vi "HostMem Reshape.vi"(4 "rows":i32, 6 "cn":i32, 8 "error in (no error)":errorcluster, 11 "HostMem in":refnum<class "HostMem.lvclass">) -> (0 "error out":errorcluster, 2 "Dst out":refnum<class "HostMem.lvclass">, 3 "HostMem out":refnum<class "HostMem.lvclass">)   [LabVIEW 2020, in "OpenLvVision_OpenCv.lvlib" / "Cuda.lvlib" / "HostMem.lvclass"]
doc: "creates alternative HostMem header for the same data, with different number of channels and/or different number of rows"
uses:
  HostMem.lvclass
  C:/Users/lukas/Downloads/OpenLvVision_OpenCv/SourceCode/LabView/OpenLvVision_OpenCv/_LvHelpers/EdvrObject/EdvrObject.lvclass
  _LvHelpers/EdvrObject/EdvrObject.lvclass/EdvrObject.ctl
  _LvHelpers/EdvrObject/TypeDef/Edvr.ctl
  OpenLvVision_OpenCv.lvlib
  <vilib>/Utility/error.llb/Error Cluster From Error Code.vi
  <vilib>/ErrorRing/Error Ring.xnode
  _LvHelpers/EdvrObject/EdvrObject.lvclass
  Dlls/OlvOpenCvWrapper.dll
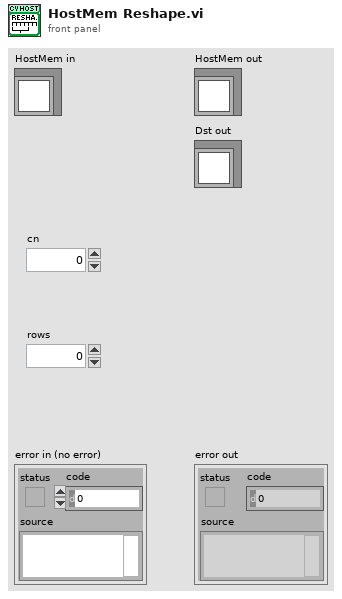
[diagram p1: front panel]
types:
  T1 = typedef "OpenLvVision_OpenCv.lvlib/EdvrObject.lvclass/Edvr.ctl" = refnum<data-value>
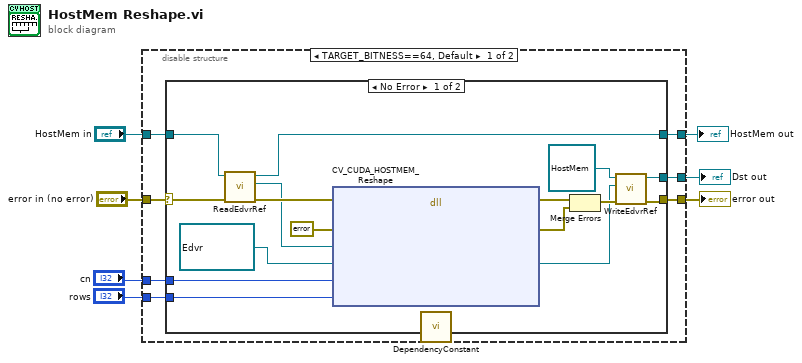
[diagram p0: block diagram]
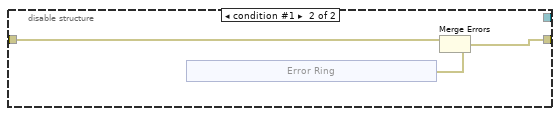
[diagram p3: hidden frame]
diagram:
  n1 = disable-structure shown="TARGET_BITNESS==64, Default" {
    disable-tunnel: "error in (no error)" -> [w14 w34]
    disable-tunnel: [w13 w35] -> w6
    disable-tunnel: "HostMem in" -> [w12 _]
    disable-tunnel: [w11 _] -> w4
    disable-tunnel: "rows" -> [w10 _]
    disable-tunnel: "cn" -> [w9 _]
    disable-tunnel: [w8 _] -> w1
    frame condition #0 (active) {
      n2 = case shown="No Error" w14 {
        selector: w14 -> [w21 w32]
        tunnel: [w18 w32] -> w13
        tunnel: w12 -> [w27 w31]
        tunnel: [w24 w31] -> w11
        tunnel: w10 -> [w23 _]
        tunnel: w9 -> [w22 _]
        tunnel: [w15 _] -> w8
        frame No Error {
          n3 = call "ReadEdvrRef.vi"("error in (no error)"=w21, "EdvrObject in"=w27) -> ("error out"=w26:errorcluster, "Edvr"=w25:T1, "EdvrObject out"=w24:refnum<class "HostMem.lvclass">)  [unwired: 7 in]
          n4 = dll-call lib="C:/Users/lukas/Downloads/OpenLvVision_OpenCv/SourceCode/LabView/OpenLvVision_OpenCv/Dlls/OlvOpenCvWrapper.dll" fn="CV_CUDA_HOSTMEM_Reshape"(error in=w26, "Error"=errorcluster {"status"=FALSE, "code"=0, "source"=""} ("error out"), "edvrRefSrc"=w25, "edvrRefDst"=T1 refnum ("Edvr"), "cn"=w22, "rows"=w23) -> (error out=w30:errorcluster, "Error"=w29:errorcluster, "edvrRefDst"=w16:T1)  [unwired: 6 in, 1 out]
          n5 = call "DependencyConstant.vi"() -> ()  [unwired: 12 in]
          n6 = Merge Errors(w30, w29) -> (w19:errorcluster)
          n7 = call "WriteEdvrRef.vi"("error in (no error)"=w19, "Edvr"=w16, "EdvrObject in"=refnum<class "HostMem.lvclass"> refnum ("Dst out")) -> ("error out"=w18:errorcluster, "EdvrObject out"=w15:refnum<class "HostMem.lvclass">)  [unwired: 7 in]
        }
        frame Error {
        }
      }
    }
    frame condition #1 {
      n8 = xnode "Error Ring"() -> ("error out"=w33:errorcluster)
      n9 = Merge Errors(w34, w33) -> (w35:errorcluster)
    }
  }
  "error out" <- w6
  "HostMem out" <- w4
  "Dst out" <- w1
